vi "measure CE BT OOB Trigger Level.vi"(8 "error in (no error)":errorcluster, 11 "SA Measurement in":refnum<class "SA Measurement.lvclass">) -> (0 "error out":errorcluster, 3 "SA Measurement out":refnum<class "SA Measurement.lvclass">)   [LabVIEW 2023, in "Spectrum Analyzer.lvlib" / "SA Measurement.lvclass"]
uses:
  SA Measurement.lvclass
  SA Measurement.lvclass/SA Measurement.ctl
  TYPE DEFINITION/TYPE RBW and VBW Select.ctl
  Spectrum Analyzer.lvlib
  TYPE DEFINITION/TYPE Marker Peak Search Type.ctl
  Interface_Spectrum/Interface_Spectrum.lvclass
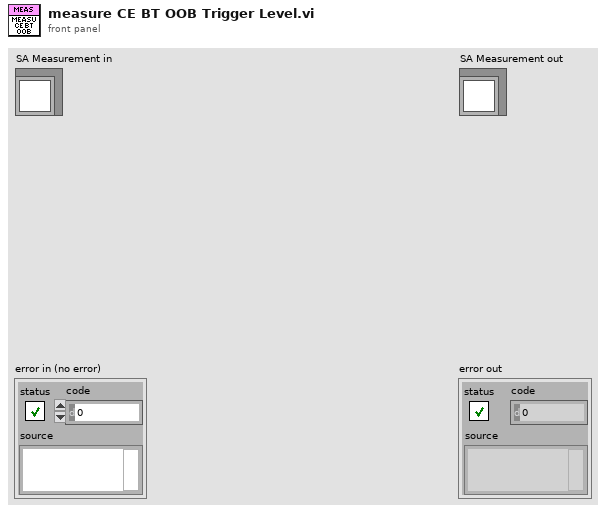
[diagram p1: front panel]
types:
  T1 = enum16{"Free Run", "Video (IF Envelop)", "RF Burst"}
  T2 = typedef "Spectrum Analyzer.lvlib/TYPE Marker Peak Search Type.ctl" = enum16{"Max", "Next Peak"}
  T3 = typedef "Spectrum Analyzer.lvlib/TYPE RBW and VBW Select.ctl" = enum16{"Res BW", "Video BW"}
  T4 = typedef "Spectrum Analyzer.lvlib/TYPE Y-axis Unit.ctl" = enum16{"dBm", "dBmV", "dBuV", "dBpW", "Volt", "Ampere", "Watt"}
  T5 = typedef "Spectrum Analyzer.lvlib/TYPE Display Trace Mode Select.ctl" = enum16{"Clear Write", "Max Hold", "Min Hold", "Average", "View"}
  T6 = typedef "Spectrum Analyzer.lvlib/TYPE Detect Mode Select.ctl" = enum16{"Det Auto (Normal)", "Auto Peak", "Positive Peak", "Negative Peak", "Sample", "RMS", "Average", "Quasipeak", "CISPR Average", "RMS Average"}
  T7 = cluster{"Trace Mode":T5, "Detector Type":T6, "Detect Auto?":bool}[]
  T8 = typedef "Spectrum Analyzer.lvlib/TYPE Marker Value.ctl" = cluster{"X-axis":dbl, "Y-axis":dbl}
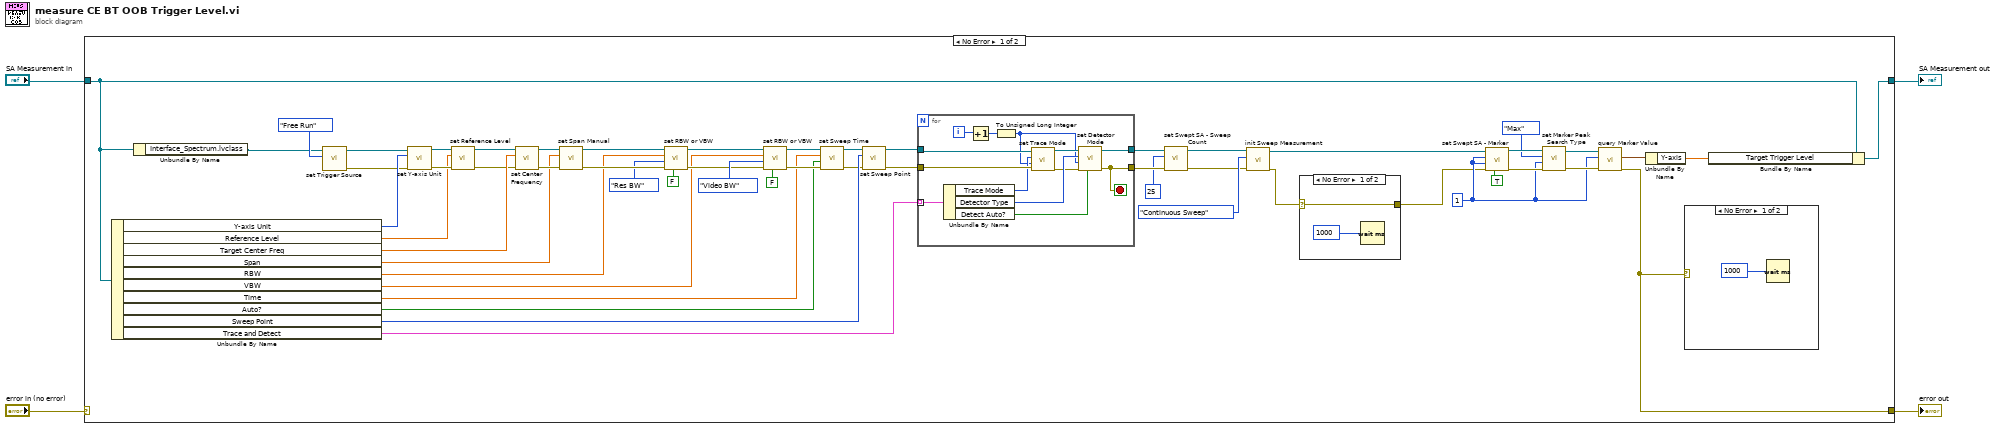
[diagram p0: block diagram]
diagram:
  n1 = case shown="No Error" "error in (no error)" {
    selector: "error in (no error)" -> [_ w78]
    tunnel: [w5 w78] -> w1
    tunnel: [w15 w77] -> w3
    tunnel: "SA Measurement in" -> [w17 w77]
    frame No Error {
      w31 = 1 ("Index")
      n2 = Unbundle By Name(w17) -> ("Y-axis Unit"=w45:T4, "Reference Level"=w28:dbl, "Target Center Freq"=w59:dbl, "Span"=w56:dbl, "RBW"=w53:dbl, "VBW"=w46:dbl, "Time"=w42:dbl, "Auto?"=w41:bool, "Sweep Point"=w25:u32, "Trace and Detect"=w40:T7)
      n3 = Unbundle By Name(w17) -> ("Interface_Spectrum.lvclass"=w8:refnum<class "Interface_Spectrum.lvclass">)
      n4 = call-dynamic "set Trigger Source.vi"("Trigger Source"=T1."Free Run", "Interface_Spectrum in"=w8) -> ("error out"=w6:errorcluster, "Interface_Spectrum out"=w7:refnum<class "Interface_Spectrum.lvclass">)  [unwired: 8 in]
      n5 = call-dynamic "set Y-axis Unit.vi"("error in (no error)"=w6, "Y-axis Unit"=w45, "Interface_Spectrum in"=w7) -> ("error out"=w29:errorcluster, "Interface_Spectrum out"=w30:refnum<class "Interface_Spectrum.lvclass">)  [unwired: 7 in]
      n6 = call-dynamic "set Reference Level.vi"("error in (no error)"=w29, "Reference Level"=w28, "Interface_Spectrum in"=w30) -> ("error out"=w26:errorcluster, "Interface_Spectrum out"=w27:refnum<class "Interface_Spectrum.lvclass">)  [unwired: 7 in]
      n7 = call-dynamic "set Center Frequency.vi"("error in (no error)"=w26, "Center Frequency (Hz)"=w59, "Interface_Spectrum in"=w27) -> ("error out"=w57:errorcluster, "Interface_Spectrum out"=w58:refnum<class "Interface_Spectrum.lvclass">)  [unwired: 7 in]
      n8 = call-dynamic "set Span Manual.vi"("error in (no error)"=w57, "Span (Hz)"=w56, "Interface_Spectrum in"=w58) -> ("error out"=w54:errorcluster, "Interface_Spectrum out"=w55:refnum<class "Interface_Spectrum.lvclass">)  [unwired: 7 in]
      n9 = call-dynamic "set RBW or VBW.vi"("BW Auto?"=FALSE, "error in (no error)"=w54, "BW Type"=TYPE_RBW_and_VBW_Select."Res BW", "BW Value (Hz)"=w53, "Interface_Spectrum in"=w55) -> ("error out"=w47:errorcluster, "Interface_Spectrum out"=w48:refnum<class "Interface_Spectrum.lvclass">)  [unwired: 5 in]
      n10 = call-dynamic "set RBW or VBW.vi"("BW Auto?"=FALSE, "error in (no error)"=w47, "BW Type"=TYPE_RBW_and_VBW_Select."Video BW", "BW Value (Hz)"=w46, "Interface_Spectrum in"=w48) -> ("error out"=w43:errorcluster, "Interface_Spectrum out"=w44:refnum<class "Interface_Spectrum.lvclass">)  [unwired: 5 in]
      n11 = call-dynamic "set Sweep Time.vi"("error in (no error)"=w43, "Sweep Time Auto?"=w41, "Sweep Time(sec)"=w42, "Interface_Spectrum in"=w44) -> ("error out"=w23:errorcluster, "Interface_Spectrum out"=w24:refnum<class "Interface_Spectrum.lvclass">)  [unwired: 6 in]
      n12 = call-dynamic "set Sweep Point.vi"("error in (no error)"=w23, "Sweep Point"=w25, "Interface_Spectrum in"=w24) -> ("error out"=w21:errorcluster, "Interface_Spectrum out"=w22:refnum<class "Interface_Spectrum.lvclass">)  [unwired: 7 in]
      n13 = for {
        tunnel: w22 -> [w75]
        tunnel: w21 -> [w74]
        tunnel: w40 -> [w76] mode=indexing
        tunnel: [w64] -> w38
        tunnel: [w65] -> w39
        i -> [w73]
        stop <- w64 stop-if-true
        n14 = Unbundle By Name(w76) -> ("Trace Mode"=w71:T5, "Detector Type"=w69:T6, "Detect Auto?"=w66:bool)
        n15 = Increment(x=w73) -> (x+1=w72:i32)
        n16 = To Unsigned Long Integer(number=w72) -> (unsigned 32bit integer=w67:u32)
        n17 = call-dynamic "set Trace Mode.vi"("error in (no error)"=w74, "Trace Index"=w67, "Trace Mode"=w71, "Interface_Spectrum in"=w75) -> ("error out"=w68:errorcluster, "Interface_Spectrum out"=w70:refnum<class "Interface_Spectrum.lvclass">)  [unwired: 6 in]
        n18 = call-dynamic "set Detector Mode.vi"("Detect Auto?"=w66, "error in (no error)"=w68, "Trace Index"=w67, "Detector Type"=w69, "Interface_Spectrum in"=w70) -> ("error out"=w64:errorcluster, "Interface_Spectrum out"=w65:refnum<class "Interface_Spectrum.lvclass">)  [unwired: 5 in]
      }
      n19 = call-dynamic "set Swept SA - Sweep Count.vi"("error in (no error)"=w38, "Sweep Count"=u32 25, "Interface_Spectrum in"=w39) -> ("error out"=w11:errorcluster, "Interface_Spectrum out"=w13:refnum<class "Interface_Spectrum.lvclass">)  [unwired: 7 in]
      n20 = call-dynamic "init Sweep Measurement.vi"("error in (no error)"=w11, "Sweep Measurement Mode"=enum16{"Single Sweep", "Continuous Sweep"}."Continuous Sweep", "Interface_Spectrum in"=w13) -> ("error out"=w12:errorcluster, "Interface_Spectrum out"=w10:refnum<class "Interface_Spectrum.lvclass">)  [unwired: 7 in]
      n21 = case shown="No Error" w12 {
        selector: w12 -> [w61 w63]
        tunnel: [w61 w63] -> w19
        frame No Error {
          n22 = Wait (ms)(milliseconds to wait=u32 1000) -> ()  [unwired: 1 out]
        }
        frame Error {
        }
      }
      n23 = call-dynamic "set Swept SA - Marker.vi"("On?"=TRUE, "error in (no error)"=w19, "trace"=w31, "Index"=w31, "Interface_Spectrum in"=w10) -> ("error out"=w35:errorcluster, "Interface_Spectrum out"=w36:refnum<class "Interface_Spectrum.lvclass">)  [unwired: 5 in]
      n24 = call-dynamic "set Marker Peak Search Type.vi"("error in (no error)"=w35, "Marker Index"=w31, "Peak Search Type"=TYPE_Marker_Peak_Search_Type."Max", "Interface_Spectrum in"=w36) -> ("error out"=w32:errorcluster, "Interface_Spectrum out"=w33:refnum<class "Interface_Spectrum.lvclass">)  [unwired: 6 in]
      n25 = call-dynamic "query Marker Value.vi"("error in (no error)"=w32, "Marker Index"=w31, "Interface_Spectrum in"=w33) -> ("error out"=w5:errorcluster, "Marker Value"=w18:T8)  [unwired: 6 in, 1 out]
      n26 = Unbundle By Name(w18) -> ("Y-axis"=w16:dbl)
      n27 = case shown="No Error" w5 {
        frame No Error {
          n28 = Wait (ms)(milliseconds to wait=u32 1000) -> ()  [unwired: 1 out]
        }
        frame Error {
        }
      }
      n29 = Bundle By Name(cluster=w17, "Target Trigger Level"=w16) -> (w15:refnum<class "SA Measurement.lvclass">)
    }
    frame Error {
    }
  }
  "error out" <- w1
  "SA Measurement out" <- w3
